vi "RemoteVI Plain Popup Click.vi"(0 "hWnd":u64, 1 "popup since":u32, 5 "window":T1, 7 "point":cluster{"x":i32, "y":i32}, 9 "posts":cluster{"msg":u32, "wParam":u64, "lParam":i64}[](array[cluster]), 11 "error in":errorcluster) -> (15 "error out":errorcluster)   [LabVIEW 2020, in "RemoteVI.lvlib"]
doc: "Clicks into a LabVIEW popup that takes no keys (colour picker, line width popup of a plot legend, graph palette popups, drop-downs) WITHOUT moving the host cursor: LabVIEW hit-tests such a click with the real cursor position (GetCursorPos) against the window's real position, and ignores posted coordinates (measured). So only the clicked window is moved, by d = real cursor - clicked point, from the window's ACTUAL position (window, listed fresh by the caller), which puts the clicked point under the host cursor; RemoteVI Post At Cursor.vi posts a WM_MOUSEMOVE and the message(s) with the cursor position as lParam, each waiting until LabVIEW has handled it; and if the window is still open afterwards it is moved back to where LabVIEW put it. So no other popup ever moves, and between messages every window is at its natural place - the OVERLAY shows it where LabVIEW shows it locally, and a submenu LabVIEW opens later opens beside an unmoved parent. A down and its up are each moved and moved back (measured with the line width popup: the width is chosen). The click waits until the popup is 350 ms old (RemoteVI Wait Popup Age.vi). No VI Server call."
uses:
  RemoteVI.lvlib
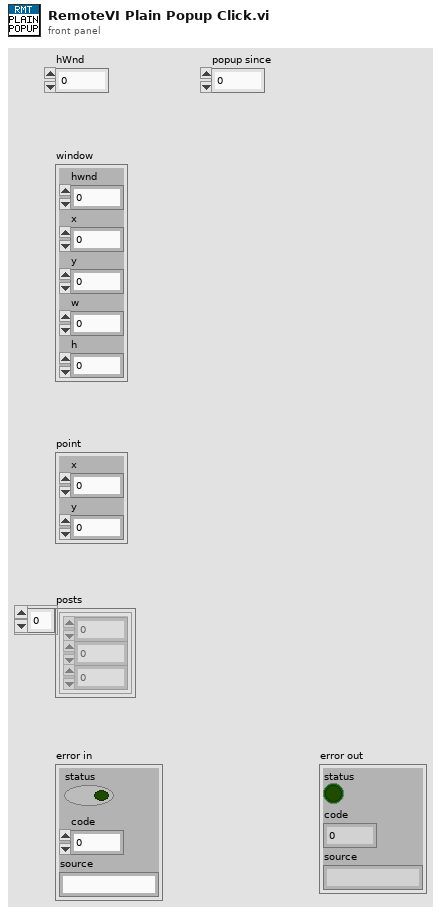
[diagram p1: front panel]
types:
  T1 = cluster{"hwnd":u64, "x":i32, "y":i32, "w":i32, "h":i32}
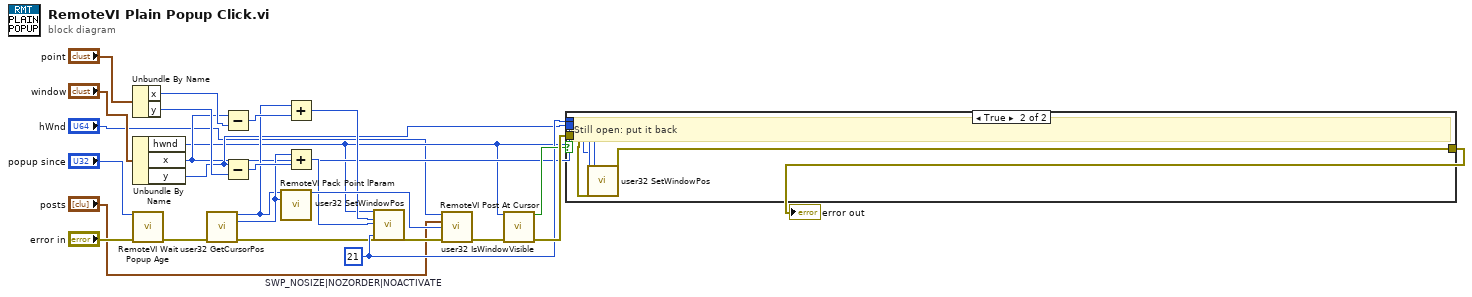
[diagram p0: block diagram]
diagram:
  w20 = u32 21  # SWP_NOSIZE|NOZORDER|NOACTIVATE
  n1 = Unbundle By Name("point") -> ("x"=w11:i32, "y"=w12:i32)
  n2 = Unbundle By Name("window") -> ("hwnd"=w8:u64, "x"=w9:i32, "y"=w10:i32)
  n3 = call "RemoteVI Wait Popup Age.vi"("popup since"="popup since", "error in"="error in") -> ("error out"=w7:errorcluster)  [unwired: 13 in]
  n4 = call "user32 GetCursorPos.vi"("error in"=w7) -> ("X"=w13:i32, "Y"=w14:i32, "error out"=w15:errorcluster)  [unwired: 11 in, 1 out]
  n5 = Subtract(x=w9, y=w11) -> (x-y=w16:i32)
  n6 = Subtract(x=w10, y=w12) -> (x-y=w17:i32)
  n7 = call "RemoteVI Pack Point lParam.vi"("x"=w13, "y"=w14) -> ("lParam"=w22:i64)  [unwired: 13 in]
  n8 = Add(x=w13, y=w16) -> (x+y=w18:i32)
  n9 = Add(x=w14, y=w17) -> (x+y=w19:i32)
  n10 = call "user32 SetWindowPos.vi"("hWnd"=w8, "X"=w18, "Y"=w19, "uFlags"=w20, "error in"=w15) -> ("error out"=w21:errorcluster)  [unwired: 21 in, 1 out]
  n11 = call "RemoteVI Post At Cursor.vi"("hWnd"="hWnd", "posts"="posts", "lParam"=w22, "error in"=w21) -> ("error out"=w23:errorcluster)  [unwired: 11 in]
  n12 = call "user32 IsWindowVisible.vi"("hWnd"=w8, "error in"=w23) -> ("visible?"=w24:bool, "error out"=w25:errorcluster)  [unwired: 12 in]
  n13 = case shown="True" w24 {
    tunnel: w20 -> [_ w32]
    tunnel: w8 -> [_ w29]
    tunnel: w9 -> [_ w30]
    tunnel: w10 -> [_ w31]
    tunnel: w25 -> [w27 w28]
    tunnel: [w27 w33] -> w26
    frame False {
    }
    frame True {
      # "Still open: put it back"
      n14 = call "user32 SetWindowPos.vi"("hWnd"=w29, "X"=w30, "Y"=w31, "uFlags"=w32, "error in"=w28) -> ("error out"=w33:errorcluster)  [unwired: 21 in, 1 out]
    }
  }
  "error out" <- w26
